vi "SMTP Email [EXPN].vi"(8 "error in (no error)":errorcluster caption="entrée d'erreur (pas d'erreur)", 10 "address":string caption="adresse", 11 "smtp session":T1 caption="session smtp") -> (0 "error out":errorcluster caption="sortie d'erreur", 1 "reply":string caption="réponse", 2 "reply code":i32 caption="code de réponse", 3 "smtp session out":T1 caption="session smtp en sortie", 4 "recipients":string[](array[string]) caption="destinataires")   [LabVIEW 2022 SP3, in "Copie de NI_SMTPEmail.lvlib"]
doc: "Envoie la commande EPN au serveur SMTP via la connexion TCP décrite par \"ID de connexion\", reçoit la réponse et l'interprète.\n\nadresse : adresse ou liste d'adresses que vous voulez étendre.\n\nCe VI renvoie \"ID de connexion en sortie\" et les résultats d'interprétation de l'erreur dans le cluster de \"sortie d'erreur\"."
uses:
  Copie de NI_SMTPEmail.lvlib
  SMTP Email Session.ctl
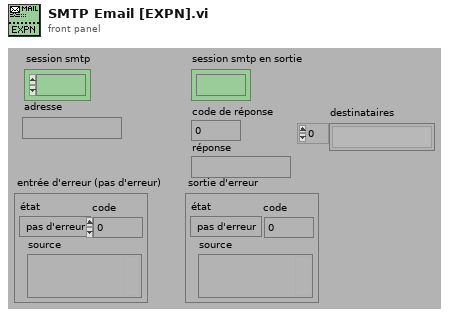
[diagram p1: front panel]
types:
  T1 = typedef "Copie de NI_SMTPEmail.lvlib/SMTP Email Session.ctl" = refnum<k1>
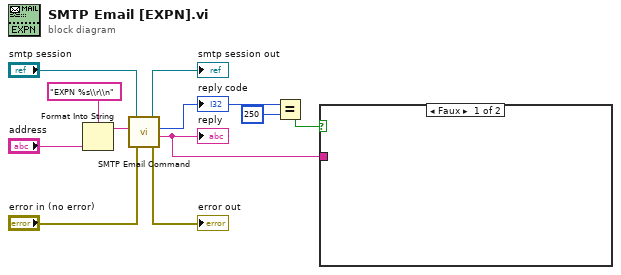
[diagram p0: block diagram]
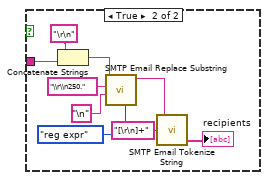
[diagram p2: hidden frame]
diagram:
  n1 = Format Into String(format string="EXPN %s\\r\\n", "address") -> (resulting string=w6:string)  [unwired: 2 in, 1 out]
  n2 = call "SMTP Email Command.vi"("error in (no error)"="error in (no error)", "command"=w6, "smtp session"="smtp session") -> ("error out"=→"error out":errorcluster, "reply"=w4:string, "reply code"=w3:i32, "smtp session out"=→"smtp session out":T1)  [unwired: 1 in]
  "reply code" <- w3
  "reply" <- w4
  n3 = Equal?(x=w3, y=250) -> (x = y?=w1:bool)
  n4 = case shown="Faux" w1 {
    tunnel: w4 -> [_ w15]
    frame False {
    }
    frame True {
      n5 = Concatenate Strings("\r\n", w15) -> (w18:string)
      n6 = call "SMTP Email Replace Substring.vi"("mode (literal)"=enum16{"literal", "wild card", "reg expr"}."reg expr", "replacement"="\n", "pattern"="\\r\\n250.", "text"=w18) -> ("text out"=w19:string)  [unwired: 6 in, 1 out]
      n7 = call "SMTP Email Tokenize String.vi"("delimiter ([\\s\\t\\n\\r]+)"="[\r\n]+" ("delimiter ([\\s\\t\\n\\r]+)"), "input string"=w19) -> ("token array"=→"recipients":string[])  [unwired: 2 in, 1 out]
    }
  }
